vi "Event_Log_Append.vi"(8 "error in (no error)":errorcluster={"status"=FALSE, "code"=0, "source"="\"\""}, 11 "State transition/command/fault details":string) -> (0 "error out":errorcluster={"status"=FALSE, "code"=0, "source"="\"\""}, 2 "status ok":bool, 3 "EventRecord enqueue status":string)   [LabVIEW 2026]
doc: "INTENT: Publish standard trace event. LOGIC: Stamp run/step/cycle IDs, monotonic event ordinal and wall-clock time; enqueue to logger."
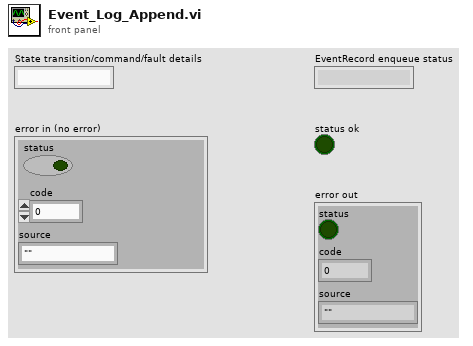
[diagram p1: front panel]
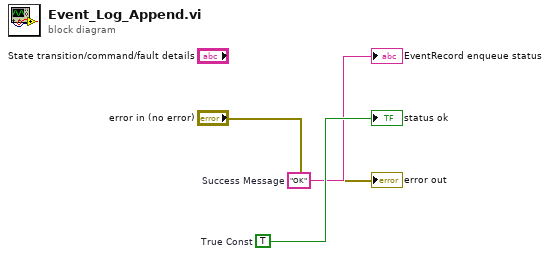
[diagram p0: block diagram]
diagram:
  w3 = TRUE  # True Const
  w2 = "OK"  # Success Message
  "EventRecord enqueue status" <- w2
  "status ok" <- w3
  "error out" <- "error in (no error)"
